vi "AddNoise.vi"(9 "Level (%)":dbl, 10 "Signal Amplitude":dbl, 11 "Signal In":dbl[](array[numeric])) -> (3 "Signal Out":dbl[](array[numeric]))   [LabVIEW 2016]
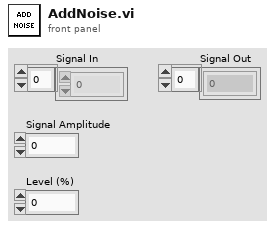
[diagram p1: front panel]
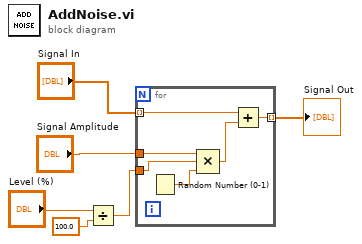
[diagram p0: block diagram]
diagram:
  n1 = Divide(x="Level (%)", y=100.0 ("x")) -> (x/y=w1:dbl)
  n2 = for {
    tunnel: "Signal In" -> [w9] mode=indexing
    tunnel: "Signal Amplitude" -> [w12]
    tunnel: w1 -> [w10]
    tunnel: [w7] -> w6 mode=indexing
    n3 = Random Number (0-1)() -> (number: 0 to 1=w11:dbl)
    n4 = Compound Arithmetic op=MULTIPLY(w12, w10, w11) -> (w8:dbl)
    n5 = Add(x=w9, y=w8) -> (x+y=w7:dbl)
  }
  "Signal Out" <- w6
